vi "Write FCC Part15c Integration BE Setting.vi"(8 "error in (no error)":errorcluster, 10 "Cluster":T1={"Window"=enum."Spectrum 1", "Start/Stop Frequency(Hz)"={"Start"=0.0, "Stop"=0.0}, "Ref"=0.0, "Atten"=0, "RBW(Hz)"=0.0, "VBW(Hz)"=0.0, "Sweep Time(sec)"=0.0, "Sweep Time Auto?"=FALSE, "Sweep Count"=0, "Sweep Point"=0, "Trace/Det"=[], "ACLR Param"={"Bandwidth"=0.0, "Offset"=0.0, "Tx Channel Count"=1}, "Center and Span Frequency(Hz)"={"Center"=0.0, "Span"=0.0}, "Frequency Line (Hz)"={"Line 1"=0.0, "Line 2"=0.0, "Activate Line1?"=FALSE, "Activate Line2?"=FALSE}} {"ACLR Param"."Tx Channel Count" min=1; "ACLR Param"."Offset" format="%#_6p"; "ACLR Param"."Bandwidth" format="%#_6p"; "Frequency Line (Hz)"."Line 2" format="%#_6p"; "Frequency Line (Hz)"."Line 1" format="%#_6p"; "Center and Span Frequency(Hz)"."Span" format="%#_6p"; "Center and Span Frequency(Hz)"."Center" format="%#_6p"; "Sweep Time(sec)" format="%#_6p"; "VBW(Hz)" format="%#_6p"; "RBW(Hz)" format="%#_6p"; "Start/Stop Frequency(Hz)"."Stop" format="%#_6p"; "Start/Stop Frequency(Hz)"."Start" format="%#_6p"}, 11 "Band Edge in":refnum<class "Band Edge.lvclass">) -> (0 "error out":errorcluster, 3 "Band Edge out":refnum<class "Band Edge.lvclass">)   [LabVIEW 2023, in "Spectrum Analyzer.lvlib" / "Band Edge.lvclass"]
uses:
  Band Edge.lvclass
  Band Edge.lvclass/Band Edge.ctl
  TYPE DEFINITION/TYPE Start and Stop Frequency.ctl
  Spectrum Analyzer.lvlib
  TYPE DEFINITION/TYPE Display Trace Mode Select.ctl
  TYPE DEFINITION/TYPE Detect Mode Select.ctl
  TYPE DEFINITION/TYPE Center and Span Frequency.ctl
  TYPE DEFINITION/TYPE Frequency Line Param.ctl
  TYPE DEFINITION/TYPE Spectrum Window Select.ctl
  TYPE DEFINITION/TYPE ACLR Setting Param.ctl
  TYPE DEFINITION/TYPE FCC Part15c Integration BandEdge Setting Cluster.ctl
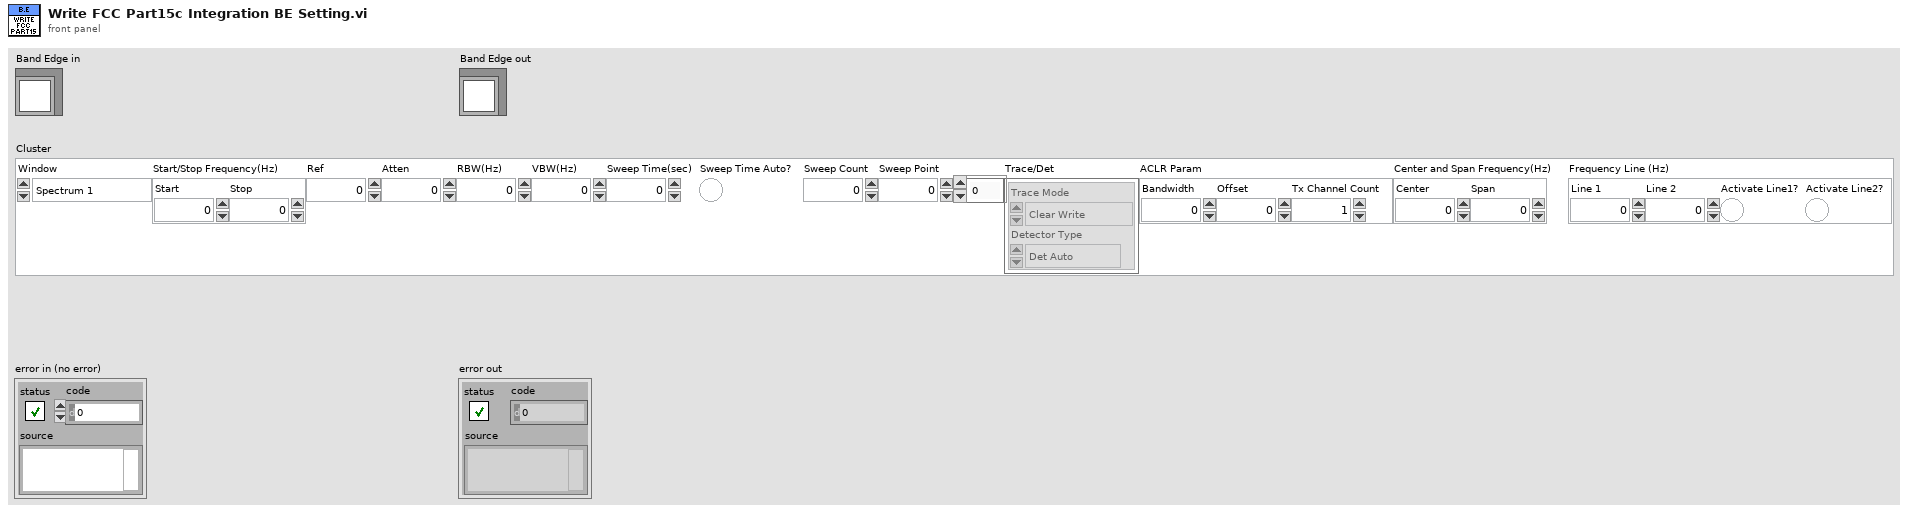
[diagram p1: front panel]
types:
  T1 = typedef "Spectrum Analyzer.lvlib/TYPE FCC Part15c Integration BandEdge Setting Cluster.ctl" = cluster{"Window":T2, "Start/Stop Frequency(Hz)":T3, "Ref":dbl, "Atten":i32, "RBW(Hz)":dbl, "VBW(Hz)":dbl, "Sweep Time(sec)":dbl, "Sweep Time Auto?":bool, "Sweep Count":u32, "Sweep Point":u32, "Trace/Det":cluster{"Trace Mode":T4, "Detector Type":T5}[], "ACLR Param":T6, "Center and Span Frequency(Hz)":T7, "Frequency Line (Hz)":T8}
  T2 = typedef "Spectrum Analyzer.lvlib/TYPE Spectrum Window Select.ctl" = enum16{"Spectrum 1", "Spectrum 2", "Spectrum 3", "Spectrum 4"}
  T3 = typedef "Spectrum Analyzer.lvlib/TYPE Start and Stop Frequency.ctl" = cluster{"Start":dbl, "Stop":dbl}
  T4 = typedef "Spectrum Analyzer.lvlib/TYPE Display Trace Mode Select.ctl" = enum16{"Clear Write", "Max Hold", "Min Hold", "Average", "View"}
  T5 = typedef "Spectrum Analyzer.lvlib/TYPE Detect Mode Select.ctl" = enum16{"Det Auto", "Auto Peak", "Positive Peak", "Negative Peak", "Sample", "RMS", "Average", "Quasipeak", "CISPR Average", "RMS Average"}
  T6 = typedef "Spectrum Analyzer.lvlib/TYPE ACLR Setting Param.ctl" = cluster{"Bandwidth":dbl, "Offset":dbl, "Tx Channel Count":i32}
  T7 = typedef "Spectrum Analyzer.lvlib/TYPE Center and Span Frequency.ctl" = cluster{"Center":dbl, "Span":dbl}
  T8 = typedef "Spectrum Analyzer.lvlib/TYPE Frequency Line Param.ctl" = cluster{"Line 1":dbl, "Line 2":dbl, "Activate Line1?":bool, "Activate Line2?":bool}
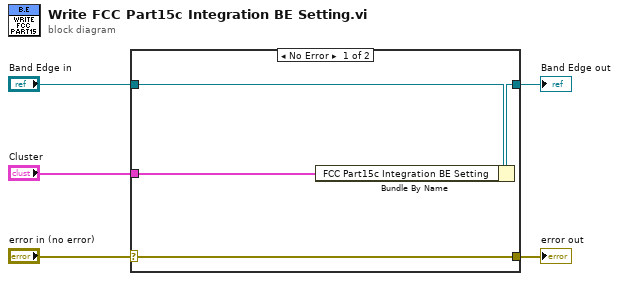
[diagram p0: block diagram]
diagram:
  n1 = case shown="No Error" "error in (no error)" {
    selector: "error in (no error)" -> [w9 w10]
    tunnel: [w9 w10] -> w4
    tunnel: [w7 w11] -> w2
    tunnel: "Band Edge in" -> [w8 w11]
    tunnel: "Cluster" -> [w6 _]
    frame No Error {
      n2 = Bundle By Name(cluster=w8, "FCC Part15c Integration BE Setting"=w6) -> (w7:refnum<class "Band Edge.lvclass">)
    }
    frame Error {
    }
  }
  "error out" <- w4
  "Band Edge out" <- w2
